vi "Variable glob alertes Keller.vi"() -> ()   [LabVIEW 2022 SP3]
panel:
  out "Groupe ON":bool[](array[boolean])
  out "Liste Keller":string[](array[string])
  in  "groupes keller":T1(array[cluster]) {"valeur alerte Keller" format="%#_6e"}
  in  "Al keller en cours":bool
  # "Alertes KELLER"
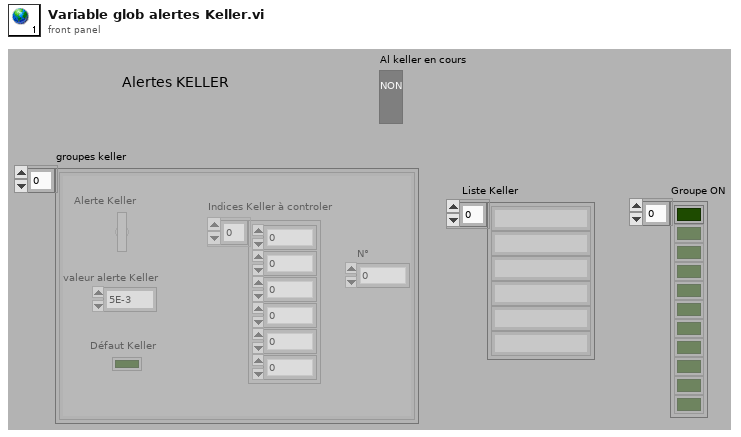
[diagram p1: front panel]
types:
  T1 = cluster{"Alerte Keller":bool, "valeur alerte Keller":dbl, "Défaut Keller":bool, "Indices Keller à controler":i16[], "N°":u16}[]
diagram:
